vi "Tank Simulator - Pump.vi"(6 "history length":i32, 7 "VC Handle":T1=-1, 8 "error in":errorcluster, 9 "cmd":enum16{"init", "get", "set"}(ring)=enum."get", 10 "state in":bool, 11 "var name":string) -> (0 "error out":errorcluster, 2 "state out":bool, 3 "var name out":string, 5 "VC Handle out":T1=-1)   [LabVIEW 2021]
doc: "Handler for <B>Pump</B> variable.\n\n::: CalcExpress Toolkit :::\nCopyright (c) 2000-2026 Konstantin Shifershteyn. All rights reserved."
uses:
  vi.lib/addons/CalcExpress/cetypes.llb/VarMan Variable Context Handle.ctl
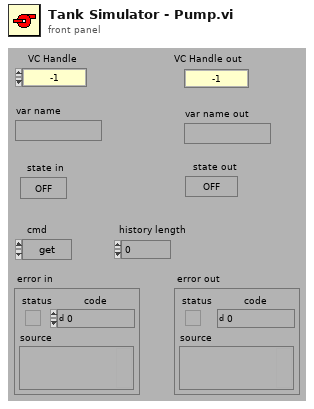
[diagram p1: front panel]
types:
  T1 = typedef "VarMan Variable Context Handle.ctl" = i32
  T2 = enum16{"create", "destroy", "set value", "get value"}
  T3 = enum32{"nop", "create", "destroy", "reset", "get info", "config"}
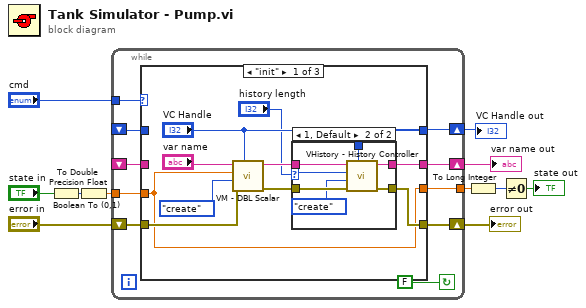
[diagram p0: block diagram]
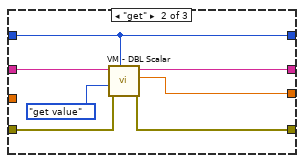
[diagram p3: hidden frame]
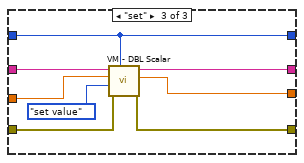
[diagram p4: hidden frame]
diagram:
  n1 = Boolean To (0,1)(Boolean="state in") -> (0, 1=w4:i16)
  n2 = To Double Precision Float(number=w4) -> (double precision float=w1:dbl)
  n3 = while {
    tunnel: [w13] -> w8
    tunnel: w1 -> [w18]
    shift-left: "error in" -> [w17]
    shift-right: [w16] -> w7
    shift-left: _ -> [w15]
    shift-right: [w20] -> w5
    shift-left: _ -> [w14]
    shift-right: [w19] -> w6
    tunnel: "cmd" -> [w21]
    stop <- FALSE continue-if-true
    n4 = case shown="\"init\"" w21 {
      tunnel: [w26 w47 w55] -> w20
      tunnel: ["VC Handle" w42 w50] -> w19
      tunnel: w18 -> [w22 _ w49]
      tunnel: w17 -> [w30 w46 w54]
      tunnel: [w23 w45 w53] -> w16
      tunnel: w15 -> [_ w43 w51]
      tunnel: w14 -> [_ w42 w50]
      tunnel: [w22 w41 w48] -> w13
      frame "init" {
        n5 = call "VM - DBL Scalar.vi"("VC Handle"="VC Handle", "error in"=w30, "cmd"=T2."create", "value in"=w22, "name_spec"="var name") -> ("error out"=w25:errorcluster, "dup name_spec"=w28:string)  [unwired: 1 in, 4 out]
        n6 = case shown="1, Default" "history length" {
          selector: "history length" -> [_ w36]
          tunnel: w28 -> [w33 w40]
          tunnel: "VC Handle" -> [_ w39]
          tunnel: [w33 w38] -> w26
          tunnel: w25 -> [w32 w37]
          tunnel: [w32 w35] -> w23
          frame 0 {
          }
          frame 1, Default {
            n7 = call "VHistory - History Controller.vi"("VC Handle"=w39, "error in"=w37, "cmd (nop:default)"=T3."create", "history length"=w36, "name_spec"=w40) -> ("error out"=w35:errorcluster, "dup name_spec"=w38:string)  [unwired: 3 in, 2 out]
          }
        }
      }
      frame "get" {
        n8 = call "VM - DBL Scalar.vi"("VC Handle"=w42, "error in"=w46, "cmd"=T2."get value", "name_spec"=w43) -> ("error out"=w45:errorcluster, "value out"=w41:dbl, "dup name_spec"=w47:string)  [unwired: 2 in, 3 out]
      }
      frame "set" {
        n9 = call "VM - DBL Scalar.vi"("VC Handle"=w50, "error in"=w54, "cmd"=T2."set value", "value in"=w49, "name_spec"=w51) -> ("error out"=w53:errorcluster, "value out"=w48:dbl, "dup name_spec"=w55:string)  [unwired: 1 in, 3 out]
      }
    }
  }
  "error out" <- w7
  "VC Handle out" <- w6
  "var name out" <- w5
  n10 = To Long Integer(number=w8) -> (32bit integer=w3:i32)
  n11 = Not Equal To 0?(x=w3) -> (x != 0?=→"state out":bool)
